vi "RemoteVI Share Rows.vi"(0 "status":T1(array[cluster])) -> (4 "items":string[][](array[string]), 5 "ports":u16[](array[numeric]))   [LabVIEW 2020, in "RemoteVI.lvlib"]
doc: "RemoteVI Server's list of hosted shares: one listbox row per share of status (RemoteVI Status.vi) - shared (target and kind), port, reach (this computer or whole network, and view only) and clients (their number, or stopped when the share's loop no longer runs) - and the ports. Pure."
uses:
  RemoteVI.lvlib
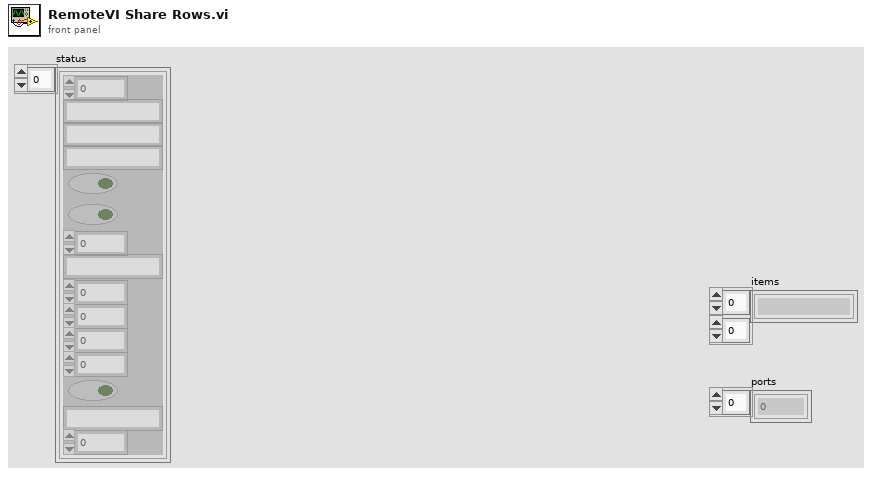
[diagram p1: front panel]
types:
  T1 = cluster{"port":u16, "url":string, "target":string, "kind":string, "whole network":bool, "running":bool, "uptime s":dbl, "clients":cluster{"address":string, "connected s":dbl, "idle s":dbl}[], "fps":dbl, "kB per s":dbl, "frames":u32, "latency ms":dbl, "view only":bool, "last error":string, "hWnd":u64}[]
  T2 = cluster{"address":string, "connected s":dbl, "idle s":dbl}[]
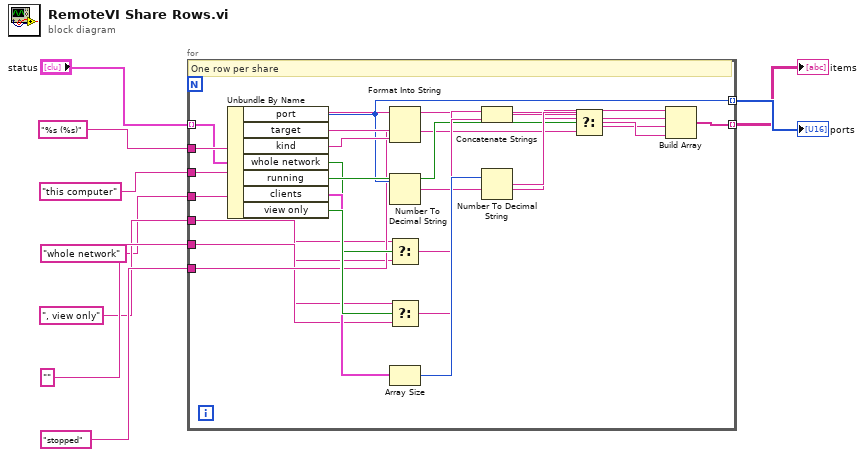
[diagram p0: block diagram]
diagram:
  n1 = for {
    tunnel: "status" -> [w10] mode=indexing
    tunnel: "%s (%s)" -> [w11]
    tunnel: "this computer" -> [w12]
    tunnel: "whole network" -> [w13]
    tunnel: ", view only" -> [w14]
    tunnel: "" -> [w15]
    tunnel: "stopped" -> [w16]
    tunnel: [w17] -> w9 mode=indexing
    tunnel: [w32] -> w8 mode=indexing
    # "One row per share"
    n2 = Unbundle By Name(w10) -> ("port"=w17:u16, "target"=w18:string, "kind"=w19:string, "whole network"=w20:bool, "running"=w21:bool, "clients"=w22:T2, "view only"=w23:bool)
    n3 = Format Into String(format string=w11, w18, w19) -> (resulting string=w24:string)  [unwired: 2 in, 1 out]
    n4 = Number To Decimal String(number=w17) -> (decimal integer string=w25:string)  [unwired: 1 in]
    n5 = Select(t=w13, s=w20, f=w12) -> (s? t:f=w26:string)
    n6 = Select(t=w14, s=w23, f=w15) -> (s? t:f=w27:string)
    n7 = Array Size(array=w22) -> (size(s)=w29:i32)
    n8 = Concatenate Strings(w26, w27) -> (w28:string)
    n9 = Number To Decimal String(number=w29) -> (decimal integer string=w30:string)  [unwired: 1 in]
    n10 = Select(t=w30, s=w21, f=w16) -> (s? t:f=w31:string)
    n11 = Build Array(w24, w25, w28, w31) -> (w32:string[])
  }
  "items" <- w8
  "ports" <- w9
